vi "SetHeaderVariantData.vi"(8 "error in (no error)":errorcluster, 9 "Value":string, 10 "Name":string, 11 "Variant in":variant) -> (0 "error out":errorcluster, 3 "Variant out":variant)   [LabVIEW 2021, in "LV WebSockets.lvlib"]
doc: "Sets a variant attribute. If the attribute already exists, it builds a comma separated string of the values (useful for keep array data).\nWebSockets 1.6.0.22\nSam Sharp - MediaMongrels Ltd\nCopyright (c) 2016, MediaMongrels Ltd"
uses:
  LV WebSockets.lvlib
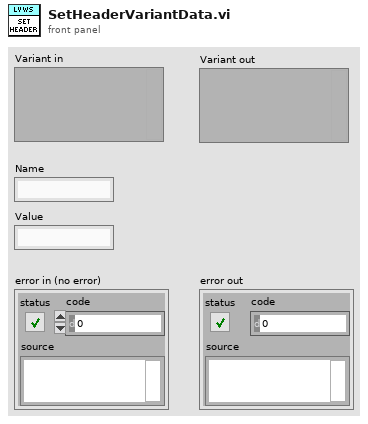
[diagram p1: front panel]
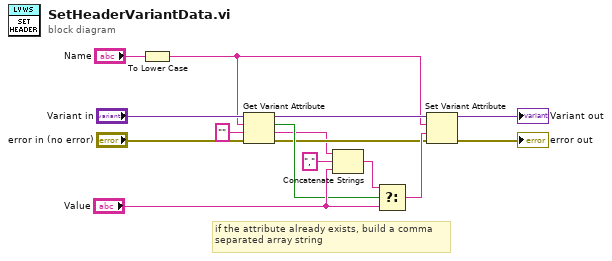
[diagram p0: block diagram]
diagram:
  # "if the attribute already exists, build a comma\nseparated array string"
  n1 = To Lower Case(string="Name") -> (all lower case string=w1:string)
  n2 = Get Variant Attribute(Variant="Variant in", name=w1, default value (empty Variant)="", error in="error in (no error)") -> (duplicate Variant=w6:variant, found=w8:bool, value=w4:string, error out=w5:errorcluster)
  n3 = Concatenate Strings(w4, "," ("string"), "Value") -> (w2:string)
  n4 = Select(t=w2, s=w8, f="Value") -> (s? t:f=w7:string)
  n5 = Set Variant Attribute(Variant=w6, name=w1, value=w7, error in=w5) -> (Variant out=→"Variant out":variant, error out=→"error out":errorcluster)  [unwired: 1 out]
